vi "BCryptGenRandom Wrapper Template.vi"(0 "byte count":u32=16, 5 "hAlgorithm":u64, 7 "dwFlags":u32=2, 11 "error in":errorcluster) -> (4 "random bytes":u8[](array[numeric]), 6 "return value":i32, 15 "error out":errorcluster)   [LabVIEW 2020]
doc: "Fills byte count bytes with cryptographically secure random numbers through bcrypt.dll BCryptGenRandom (stdcall, called in any thread) with the system-preferred random number generator (hAlgorithm NULL, dwFlags BCRYPT_USE_SYSTEM_PREFERRED_RNG = 2). return value is the NTSTATUS: 0 on success. When error in carries an error the DLL is not called. Generated by scripts\\Build Win32 Wrappers.vi - do not edit by hand, rebuild it."
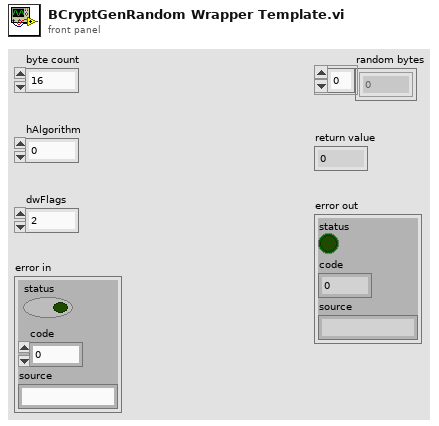
[diagram p1: front panel]
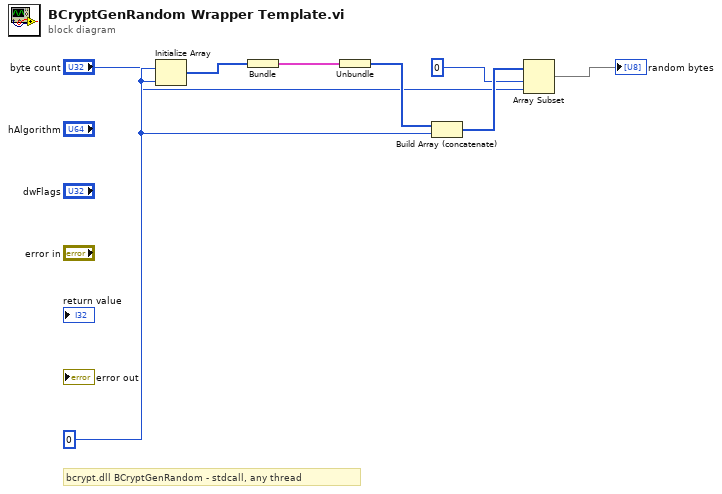
[diagram p0: block diagram]
diagram:
  w3 = u8 0
  # "bcrypt.dll BCryptGenRandom - stdcall, any thread"
  n1 = Initialize Array(w3, "byte count") -> (w5:u8[])
  n2 = Bundle(w5) -> (w6:cluster{u8[]})  [unwired: 1 in]
  n3 = Unbundle(w6) -> (w7:u8[])
  n4 = Build Array (concatenate)(w7, w3) -> (w8:u8[])
  n5 = Array Subset(array=w8, index=0, length="byte count") -> (→"random bytes":u8[])
